vi "Set Turn Table Param.vi"(8 "error in (no error)":errorcluster, 10 "Turn Table Info":T1, 11 "AUDIX EM1000 in":refnum<class "AUDIX EM1000.lvclass">) -> (0 "error out":errorcluster, 3 "AUDIX EM1000 out":refnum<class "AUDIX EM1000.lvclass">)   [LabVIEW 2023, in "Turn Table and Mast.lvlib" / "AUDIX EM1000.lvclass"]
uses:
  AUDIX EM1000.lvclass
  AUDIX EM1000.lvclass/AUDIX EM1000.ctl
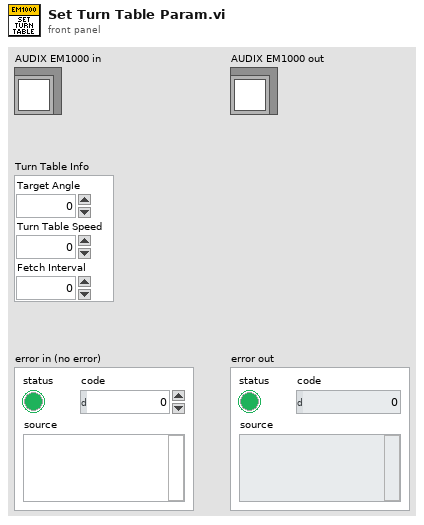
[diagram p1: front panel]
types:
  T1 = cluster{"Target Angle":i32, "Turn Table Speed":i32, "Fetch Interval":i32}
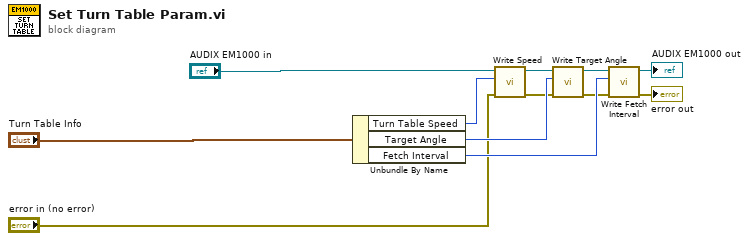
[diagram p0: block diagram]
diagram:
  n1 = Unbundle By Name("Turn Table Info") -> ("Turn Table Speed"=w10:i32, "Target Angle"=w11:i32, "Fetch Interval"=w12:i32)
  n2 = call "Write Speed.vi"("error in (no error)"="error in (no error)", "Speed"=w10, "AUDIX EM1000 in"="AUDIX EM1000 in") -> ("error out"=w4:errorcluster, "AUDIX EM1000 out"=w3:refnum<class "AUDIX EM1000.lvclass">)  [unwired: 7 in]
  n3 = call "Write Target Angle.vi"("error in (no error)"=w4, "Target Angle"=w11, "AUDIX EM1000 in"=w3) -> ("error out"=w6:errorcluster, "AUDIX EM1000 out"=w5:refnum<class "AUDIX EM1000.lvclass">)  [unwired: 7 in]
  n4 = call "Write Fetch Interval.vi"("error in (no error)"=w6, "Fetch Interval"=w12, "AUDIX EM1000 in"=w5) -> ("error out"=→"error out":errorcluster, "AUDIX EM1000 out"=→"AUDIX EM1000 out":refnum<class "AUDIX EM1000.lvclass">)  [unwired: 7 in]
